vi "IsWindowVisible Wrapper Template.vi"(0 "hWnd":u64, 11 "error in":errorcluster) -> (4 "visible?":bool, 15 "error out":errorcluster)   [LabVIEW 2020]
doc: "TRUE when the window hWnd has the WS_VISIBLE style (it may still be covered or off screen), through user32.dll IsWindowVisible (stdcall, called in any thread). FALSE also when hWnd is not a window. When error in carries an error the DLL is not called. Generated by scripts\\Build Win32 Wrappers.vi - do not edit by hand, rebuild it."
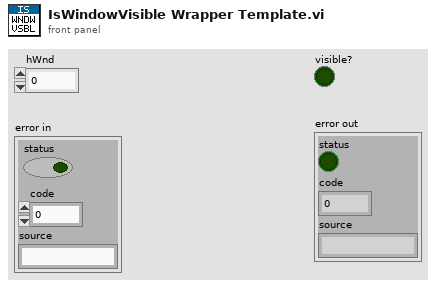
[diagram p1: front panel]
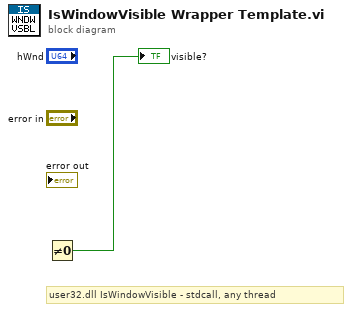
[diagram p0: block diagram]
diagram:
  # "user32.dll IsWindowVisible - stdcall, any thread"
  n1 = Not Equal To 0?() -> (x != 0?=→"visible?":bool)  [unwired: 1 in]
